vi "libssh2_channel_window_write_ex.vi"(8 "error in (no error)":errorcluster, 11 "channel":T1) -> (0 "error out":errorcluster, 2 "initial window size":u32, 3 "remaining write window":u32)   [LabVIEW 2017, in "libssh2.lvlib"]
doc: "Returns the number of bytes which may safely be written on the channel without blocking.\n\n<B>initial window size</B> returns the initial window size as defined by the channel_open request. It may be zero for locally initiated channels."
uses:
  libssh2.lvlib
  Channel Refnum.ctl
  Acquire Session.vi
  Release Session.vi
  Not A Channel.vi
  <vilib>/Utility/error.llb/Error Cluster From Error Code.vi
  Global Settings.vi
  Read Channel Refnum.vi
  Read Session Refnum.vi
  <vilib>/Utility/semaphor.llb/Acquire Semaphore.vi
  <vilib>/Utility/semaphor.llb/Release Semaphore.vi
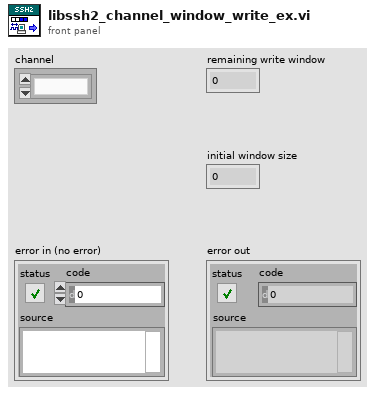
[diagram p1: front panel]
types:
  T1 = typedef "libssh2.lvlib/Channel Refnum.ctl" = refnum<k1>
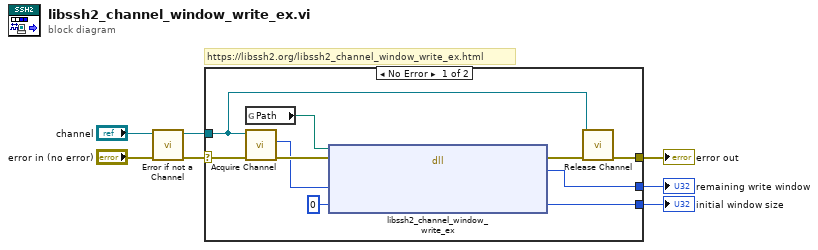
[diagram p0: block diagram]
diagram:
  # "https://libssh2.org/libssh2_channel_window_write_ex.html"
  n1 = call "Error if not a Channel.vi"("error in (no error)"="error in (no error)", "channel"="channel") -> ("error out"=w3:errorcluster, "channel out"=w1:T1)  [unwired: 8 in]
  n2 = case shown="No Error" w3 {
    selector: w3 -> [w17 w18]
    tunnel: [w9 w18] -> w7
    tunnel: w1 -> [w8 _]
    tunnel: [w15 _] -> w5
    tunnel: [w14 _] -> w4
    frame No Error {
      n3 = global read "Global Settings.vi" "Path"() -> (w11:path)
      n4 = call "Acquire Channel.vi"("error in (no error)"=w17, "channel"=w8) -> ("error out"=w13:errorcluster, "LIBSSH2_CHANNEL*"=w12:u64)  [unwired: 8 in]
      n5 = dll-call lib="?" fn="libssh2_channel_window_write_ex"(path in=w11, error in=w13, "channel"=w12, "window_size_initial"=u32 0) -> (error out=w16:errorcluster, "return value"=w14:u32, "window_size_initial"=w15:u32)  [unwired: 2 in, 1 out]
      n6 = call "Release Channel.vi"("error in (no error)"=w16, "channel"=w8) -> ("error out"=w9:errorcluster)  [unwired: 9 in]
    }
    frame Error {
    }
  }
  "error out" <- w7
  "initial window size" <- w5
  "remaining write window" <- w4
